vi "VIH Dialog - Allow_Optional_Terminals in Context Help.vi"(8 "error in":errorcluster, 10 "Force dialog (F)":bool) -> (0 "error out":errorcluster)   [LabVIEW 2014]
doc: "::: VI Helpeks :::\nCopyright (c) 2000-2026 Konstantin Shifershteyn. All rights reserved."
panel:
  in  "ShowMore":bool caption="Show how to activate this option"
  in  "%Close":bool
  # "In order to VI Helpeks can properly obtain VI Connector Pane images,\nenable the Show Optional Terminals and Full Path option in\nthe Context Help window."
  # "This window will close automatically as soon as you enable this option"
  # "Click this button in the Context Help window"
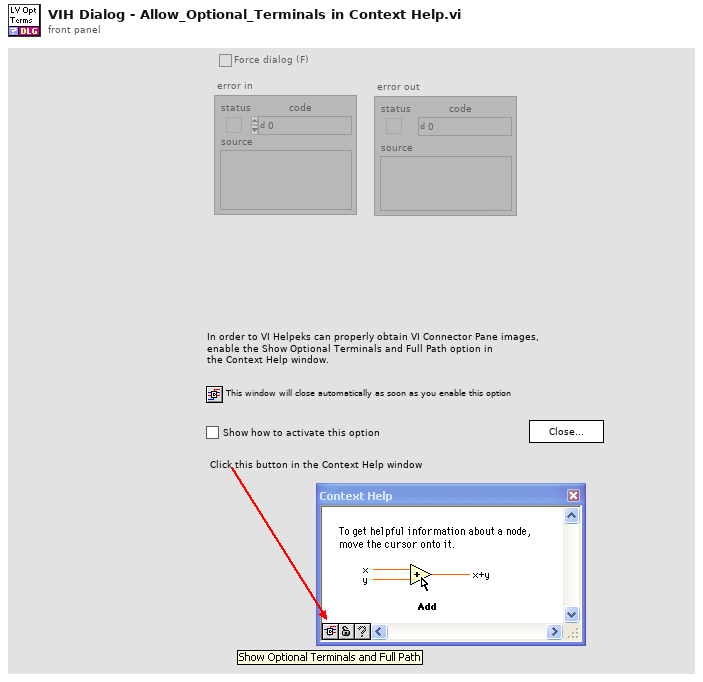
[diagram p1: front panel]
types:
  T1 = enum32{"Invalid", "Default", "Floating", "Floating/Auto-Hide", "Modal"}
  T2 = typedef "LVRectTypeDef.ctl" = cluster{"Left":i16, "Top":i16, "Right":i16, "Bottom":i16}
  T3 = typedef "LVPointTypeDef.ctl" = cluster{"Horizontal":i16, "Vertical":i16}
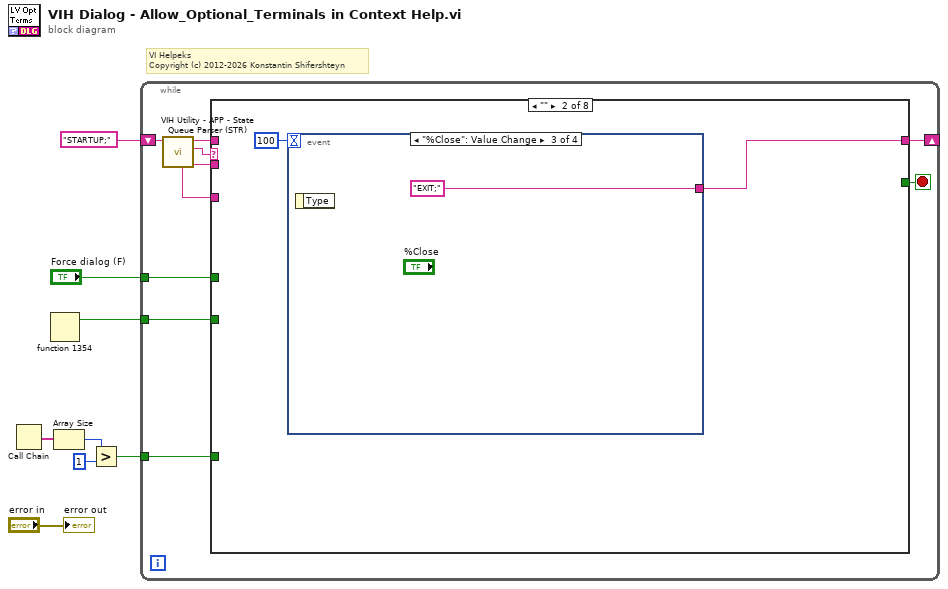
[diagram p0: block diagram]
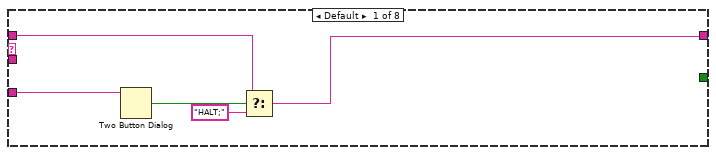
[diagram p2: hidden frame]
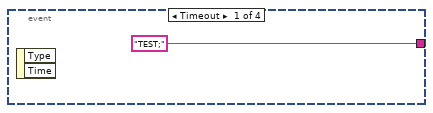
[diagram p3: hidden frame]
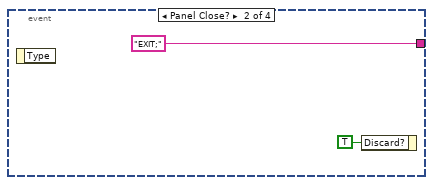
[diagram p4: hidden frame]
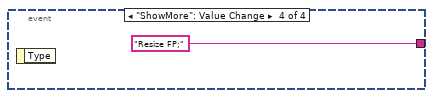
[diagram p5: hidden frame]
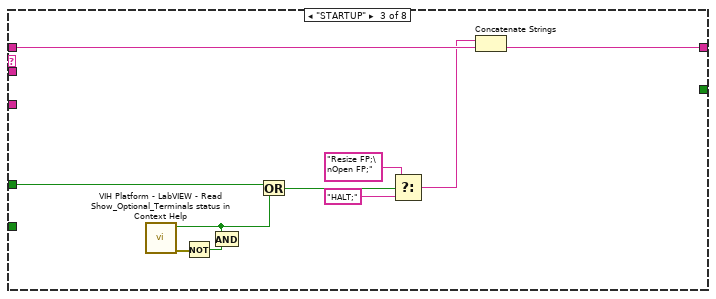
[diagram p6: hidden frame]
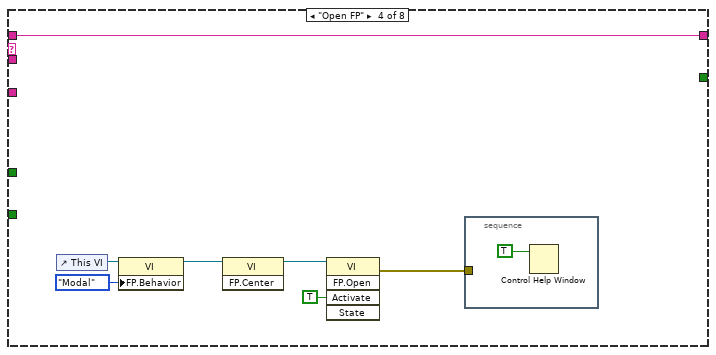
[diagram p7: hidden frame]
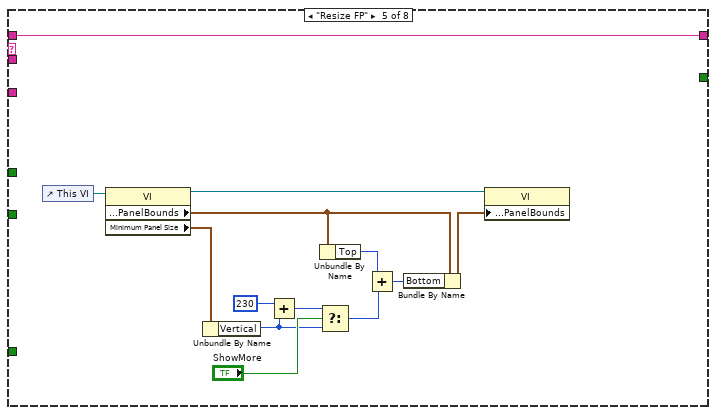
[diagram p8: hidden frame]
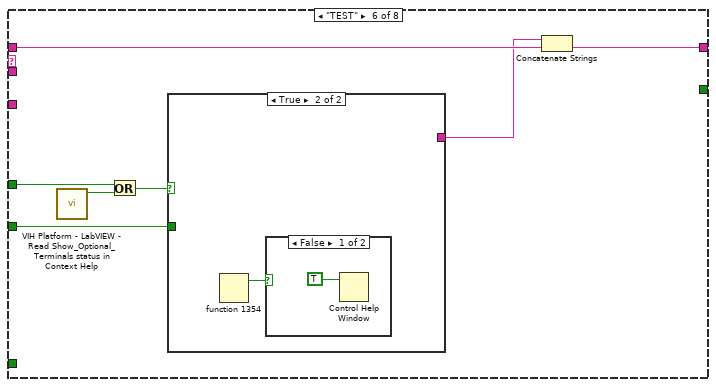
[diagram p9: hidden frame]
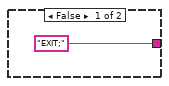
[diagram p10: hidden frame]
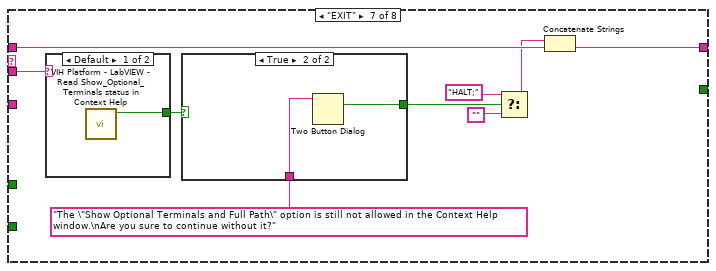
[diagram p12: hidden frame]
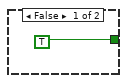
[diagram p13: hidden frame]
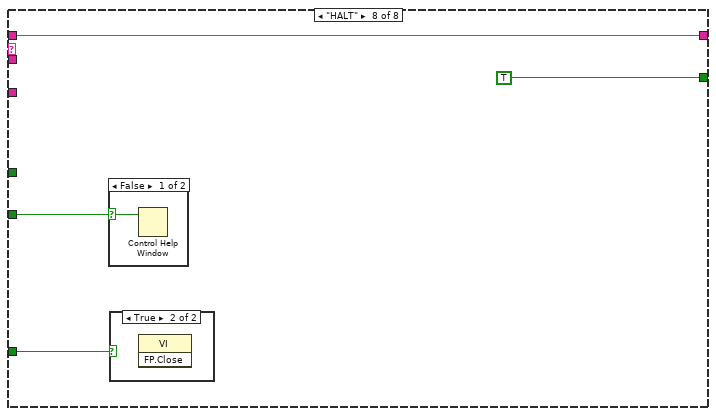
[diagram p15: hidden frame]
diagram:
  # "VI Helpeks\nCopyright (c) 2012-2026 Konstantin Shifershteyn"
  n1 = Call Chain() -> (call chain=w2:string[])
  n2 = fn#1354() -> (1:w5:bool)  [unwired: 1 out]
  n3 = Array Size(array=w2) -> (size(s)=w3:i32)
  n4 = Greater?(x=w3, y=1) -> (0:w1:bool)
  n5 = while {
    shift-right: [w16] -> _
    shift-left: "STARTUP;" -> [w18]
    tunnel: "Force dialog (F)" -> [w12]
    tunnel: w5 -> [w11]
    tunnel: w1 -> [w9]
    stop <- w13 stop-if-true
    n6 = call "VIH Utility - APP - State Queue Parser (STR).vi"("input queue"=w18) -> ("state parameters"=w10:string, "state"=w17:string, "remained queue"=w15:string, "complete state specifier"=w14:string)  [unwired: 5 in]
    n7 = case shown="\"\"" w17 {
      tunnel: [w19 w24 w39 w47 w61 w67 w79 w88] -> w16
      tunnel: w15 -> [w20 _ w40 w47 w61 w68 w80 w88]
      tunnel: w14 -> [w23 _ _ _ _ _ _ _]
      tunnel: [_ _ _ _ _ _ _ TRUE] -> w13
      tunnel: w12 -> [_ _ w34 _ _ w66 _ _]
      tunnel: w11 -> [_ _ _ _ _ w64 _ w86]
      tunnel: w10 -> [_ _ _ _ _ _ w78 _]
      tunnel: w9 -> [_ _ _ _ _ _ _ w85]
      frame Default {
        n8 = Two Button Dialog(message=w23) -> (T button?=w22:bool)  [unwired: 2 in]
        n9 = Select(t=w20, s=w22, f="HALT;") -> (s? t:f=w19:string)
      }
      frame "" {
        n10 = event shown="[2] \"%Close\": Value Change" {
          selector: _ -> [_ _ _ _]
          dyn-events: _ -> [_ _ _ _]
          timeout: 100 -> [_ _ _ _]
          tunnel: ["TEST;" "EXIT;" "EXIT;" "Resize FP;"] -> w24
          event Timeout {
            n11 = event-data() -> ()  [unwired: 1 in, 2 out]
          }
          event Panel Close? {
            n12 = event-data() -> ()  [unwired: 1 in, 1 out]
            n13 = event-data("Discard?"=TRUE) -> ()  [unwired: 1 in, 1 out]
          }
          event "%Close": Value Change {
            n14 = event-data() -> ()  [unwired: 1 in, 1 out]
          }
          event "ShowMore": Value Change {
            n15 = event-data() -> ()  [unwired: 1 in, 1 out]
          }
        }
      }
      frame "STARTUP" {
        n16 = call "VIH Platform - LabVIEW - Read Show_Optional_Terminals status in Context Help.vi"() -> ("error out"=w31:errorcluster, "simpleDiagramHelp (Hide Optional Terminals)"=w32:bool)  [unwired: 10 in]
        n17 = Not(x=w31) -> (.not. x?=w35:bool)
        n18 = And(x=w32, y=w35) -> ()  [unwired: 1 out]
        n19 = Or(x=w34, y=w32) -> (x .or. y?=w33:bool)
        n20 = Select(t="Resize FP;\nOpen FP;", s=w33, f="HALT;") -> (s? t:f=w36:string)
        n21 = Concatenate Strings(w36, w40) -> (w39:string)
      }
      frame "Open FP" {
        n22 = control-ref of="This VI"() -> (w42:refnum<vi>)
        n23 = property class="VI"(reference=w42, "FP.Behavior"=T1."Modal" ("Front Panel Window:Behavior")) -> (reference out=w45:refnum<vi>)  [unwired: 1 in, 1 out]
        n24 = invoke class="VI" method="FP.Center"(reference=w45) -> (reference out=w44:refnum<vi>)  [unwired: 2 in, 2 out]
        n25 = invoke class="VI" method="FP.Open"(reference=w44, "Activate"=TRUE ("Activate?")) -> (error out=w41:errorcluster)  [unwired: 3 in, 4 out]
        n26 = stacked-sequence {
          tunnel: w41 -> [_]
          frame #0 {
            n27 = Control Help Window(1:TRUE ("Show")) -> ()  [unwired: 1 in]
          }
        }
      }
      frame "Resize FP" {
        n28 = control-ref of="This VI"() -> (w60:refnum<vi>)
        n29 = property class="VI"(reference=w60) -> (reference out=w59:refnum<vi>, "Front Panel.PanelBounds"=w58:T2, "Minimum Panel Size"=w54:T3)  [unwired: 1 in, 1 out]
        n30 = Unbundle By Name(w54) -> ("Vertical"=w50:i16)
        n31 = Add(x=i16 230, y=w50) -> (x+y=w51:i16)
        n32 = Unbundle By Name(w58) -> ("Top"=w57:i16)
        n33 = Select(t=w51, s="ShowMore", f=w50) -> (s? t:f=w52:i16)
        n34 = Add(x=w57, y=w52) -> (x+y=w56:i16)
        n35 = Bundle By Name(cluster=w58, "Bottom"=w56) -> (w55:T2)
        n36 = property class="VI"(reference=w59, "Front Panel.PanelBounds"=w55) -> ()  [unwired: 1 in, 2 out]
      }
      frame "TEST" {
        n37 = call "VIH Platform - LabVIEW - Read Show_Optional_Terminals status in Context Help.vi"() -> ("simpleDiagramHelp (Hide Optional Terminals)"=w65:bool)  [unwired: 10 in, 1 out]
        n38 = Or(x=w66, y=w65) -> (x .or. y?=w62:bool)
        n39 = case shown="True" w62 {
          tunnel: w64 -> [_ _]
          tunnel: ["EXIT;" _] -> w63
          frame False {
          }
          frame True {
            n40 = fn#1354() -> (1:w70:bool)  [unwired: 1 out]
            n41 = case shown="False" w70 {
              frame False {
                n42 = Control Help Window(1:TRUE ("Show")) -> ()  [unwired: 1 in]
              }
              frame True {
              }
            }
          }
        }
        n43 = Concatenate Strings(w63, w68) -> (w67:string)
      }
      frame "EXIT" {
        n44 = case shown="Default" w78 {
          tunnel: [w84 _] -> w77
          frame Default {
            n45 = call "VIH Platform - LabVIEW - Read Show_Optional_Terminals status in Context Help.vi"() -> ("simpleDiagramHelp (Hide Optional Terminals)"=w84:bool)  [unwired: 10 in, 1 out]
          }
          frame "FORCE" {
          }
        }
        n46 = case shown="True" w77 {
          tunnel: [TRUE w83] -> w73
          tunnel: "The \"Show Optional Terminals and Full Path\" option is still not allowed in the Context Help window.\nAre you sure to continue without it?" -> [_ w82]
          frame False {
          }
          frame True {
            n47 = Two Button Dialog(message=w82) -> (T button?=w83:bool)  [unwired: 2 in]
          }
        }
        n48 = Select(t="HALT;" ("string"), s=w73, f="") -> (s? t:f=w74:string)
        n49 = Concatenate Strings(w74, w80) -> (w79:string)
      }
      frame "HALT" {
        n50 = case shown="False" w86 {
          selector: w86 -> [w89 _]
          frame False {
            n51 = Control Help Window(1:w89) -> ()  [unwired: 1 in]
          }
          frame True {
          }
        }
        n52 = case shown="True" w85 {
          frame False {
          }
          frame True {
            n53 = invoke class="VI" method="FP.Close"() -> ()  [unwired: 3 in, 3 out]
          }
        }
      }
    }
  }
  "error out" <- "error in"
